vi "Run.vi"(8 "error in (no error)":errorcluster, 10 "UI Refs":T1, 11 "H1 Hydraulic":refnum<class "H1 Hydraulic.lvclass">) -> (0 "error out":errorcluster, 3 "H1 Hydraulic out":refnum<class "H1 Hydraulic.lvclass">)   [LabVIEW 2025, in "H1 Plotter.lvlib" / "H1 Hydraulic.lvclass"]
uses:
  H1 Hydraulic.lvclass
  H1 Hydraulic.lvclass/H1 Hydraulic.ctl
  Users/Public/Documents/Sandia National Labs/TSS Plugin/Tests/XY Plotter.lvlibp/XY Plotter configuration/Read XY Plotter.vi
  Users/Public/Documents/Sandia National Labs/TSS Plugin/Tests/XY Plotter.lvlibp/XY  Plotter/XY Plotter.lvclass
  Users/Public/Documents/Sandia National Labs/TSS Plugin/CEF.lvlibp/serializable configuration/CEF_serializable configuration.lvclass
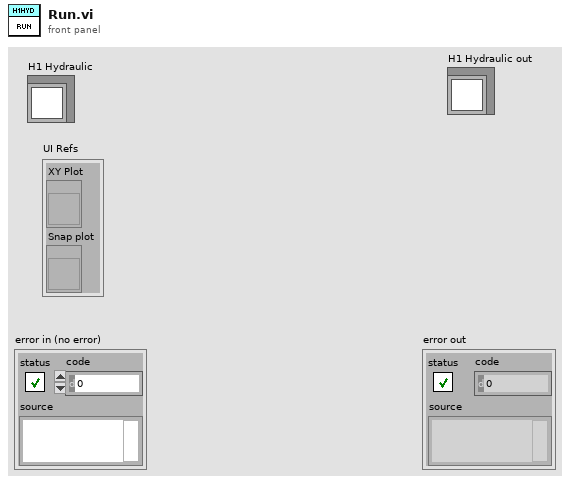
[diagram p1: front panel]
types:
  T1 = cluster{"XY Plot":refnum<vi>, "Snap plot":refnum<vi>}
  T2 = cluster{"Name":string, "Color":u32, "Style":u8, "Point Style":u8, "Name Visible":bool, "Allow Drag":bool, "Annotation Mode":u32, "Plot":i32, "Index":i32, "Position":cluster{"X":dbl, "Y":dbl}, "X Scale":u32, "Y Scale":u32, "Show Arrow":bool, "Lock Name":bool, "Plot Area":i32, "Label Offset":cluster{"X":dbl, "Y":dbl}}
  T3 = cluster{"Name":string, "Color":u32, "Style":u8, "Point Style":u8, "Name Visible":bool, "Allow Drag":bool, "Annotation Mode":u32, "Plot":i32, "Index":i32, "Position":cluster{"X":dbl, "Y":dbl}, "X Scale":u32, "Y Scale":u32, "Show Arrow":bool, "Lock Name":bool, "Plot Area":i32, "Label Offset":cluster{"X":dbl, "Y":dbl}}[]
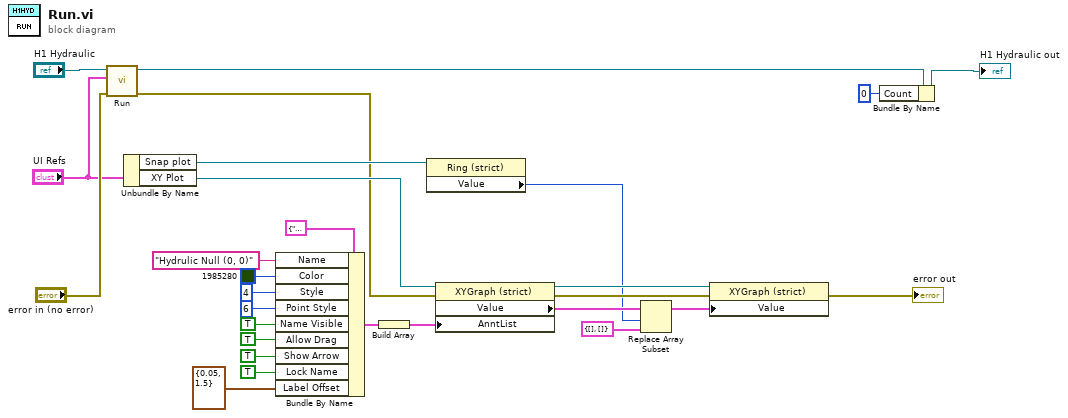
[diagram p0: block diagram]
diagram:
  n1 = call-parent "Run.vi"("error in (no error)"="error in (no error)", "UI Refs"="UI Refs", "XY Plotter"="H1 Hydraulic") -> ("error out"=w1:errorcluster, "XY Plotter out"=w28:refnum<class "H1 Hydraulic.lvclass">)  [unwired: 7 in]
  n2 = Unbundle By Name("UI Refs") -> ("Snap plot"=w3:refnum<vi>, "XY Plot"=w4:refnum<vi>)
  n3 = Bundle By Name(cluster=T2 {"Name"="", "Color"=0, "Style"=0, "Point Style"=0, "Name Visible"=FALSE, "Allow Drag"=FALSE, "Annotation Mode"=0, "Plot"=0, "Index"=0, "Position"={"X"=0.0, "Y"=0.0}, "X Scale"=0, "Y Scale"=0, "Show Arrow"=FALSE, "Lock Name"=FALSE, "Plot Area"=0, "Label Offset"={"X"=0.0, "Y"=0.0}}, "Name"="Hydrulic Null (0, 0)" ("Hydraulic Null"), "Color"=u32 1985280, "Style"=u8 4, "Point Style"=u8 6, "Name Visible"=TRUE, "Allow Drag"=TRUE, "Show Arrow"=TRUE, "Lock Name"=TRUE, "Label Offset"=cluster{"X":dbl, "Y":dbl} {"X"=0.05, "Y"=1.5}) -> (w8:T2)
  n4 = Build Array(w8) -> (w7:T3)
  n5 = property class="Ring (strict)"(reference=w3) -> ("Value"=w21:u16)  [unwired: 1 in, 2 out]
  n6 = property class="XYGraph (strict)"(reference=w4, error in=w1, "AnntList"=w7) -> (reference out=w25:refnum<vi>, error out=w26:errorcluster, "Value"=w23:cluster{"Wavenumber":dbl[], "Data":dbl[]}[])
  n7 = Replace Array Subset(array=w23, new element=cluster{"Wavenumber":dbl[], "Data":dbl[]} {"Wavenumber"=[], "Data"=[]} ("Spectrum"), index=w21) -> (w22:cluster{"Wavenumber":dbl[], "Data":dbl[]}[])
  n8 = property class="XYGraph (strict)"(reference=w25, error in=w26, "Value"=w22) -> (error out=→"error out":errorcluster)  [unwired: 1 out]
  n9 = Bundle By Name(cluster=w28, "Count"=0) -> (→"H1 Hydraulic out":refnum<class "H1 Hydraulic.lvclass">)
